vi "Scale By.vi"(0 "obj in":refnum<class "Sensor.lvclass">, 1 "Factor":dbl=1.0) -> (2 "obj out":refnum<class "Sensor.lvclass">)   [LabVIEW 2026, in "Sensor.lvclass"]
doc: "Round14: Sensor's override of Can Scale:Scale By. Same pane shape as the interface declares (obj in, Factor, obj out); the diagram is a pass-through because a class-typed unbundle cannot be authored in AIXML."
uses:
  Sensor.lvclass
  Sensor.lvclass/Sensor.ctl
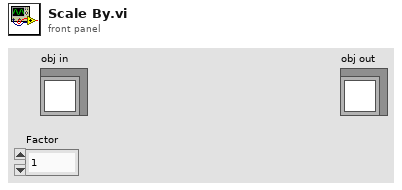
[diagram p1: front panel]
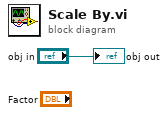
[diagram p0: block diagram]
diagram:
  "obj out" <- "obj in"
